vi "thermal_optical_capture_9.vi"() -> ()   [LabVIEW 2025]
panel:
  out "Times between Frames":u32
  in  "STOP ACQUISITION":bool
  out "File Name Out":string
  in  "File Path":string="C:\\Digambar\\Metal_thin_wall\\Optical_images\\Optical_images"
  out "Optical Preview":T1(plugin-control)
  in  "Focus":dbl(slide) scale=0.0..100.0
  out "Thermal Frame Out":string
  in  "Thermal Output Folder":path
  in  "thermal capture interval (s)":dbl
  in  "Flag Button":bool
  in  "Stop & Save":bool
  in  "Record":bool
  # "(1) Run VI"
  # "(2) After thermal camera calibration message (in terminal), press START"
  # "(3) Stop & Save"
  # "THERMAL CONTROLS"
  # "(Enter \"28\")"
  # "Thermal Record"
  # "OPTICAL CONTROLS"
  # "(must be an empty folder)"
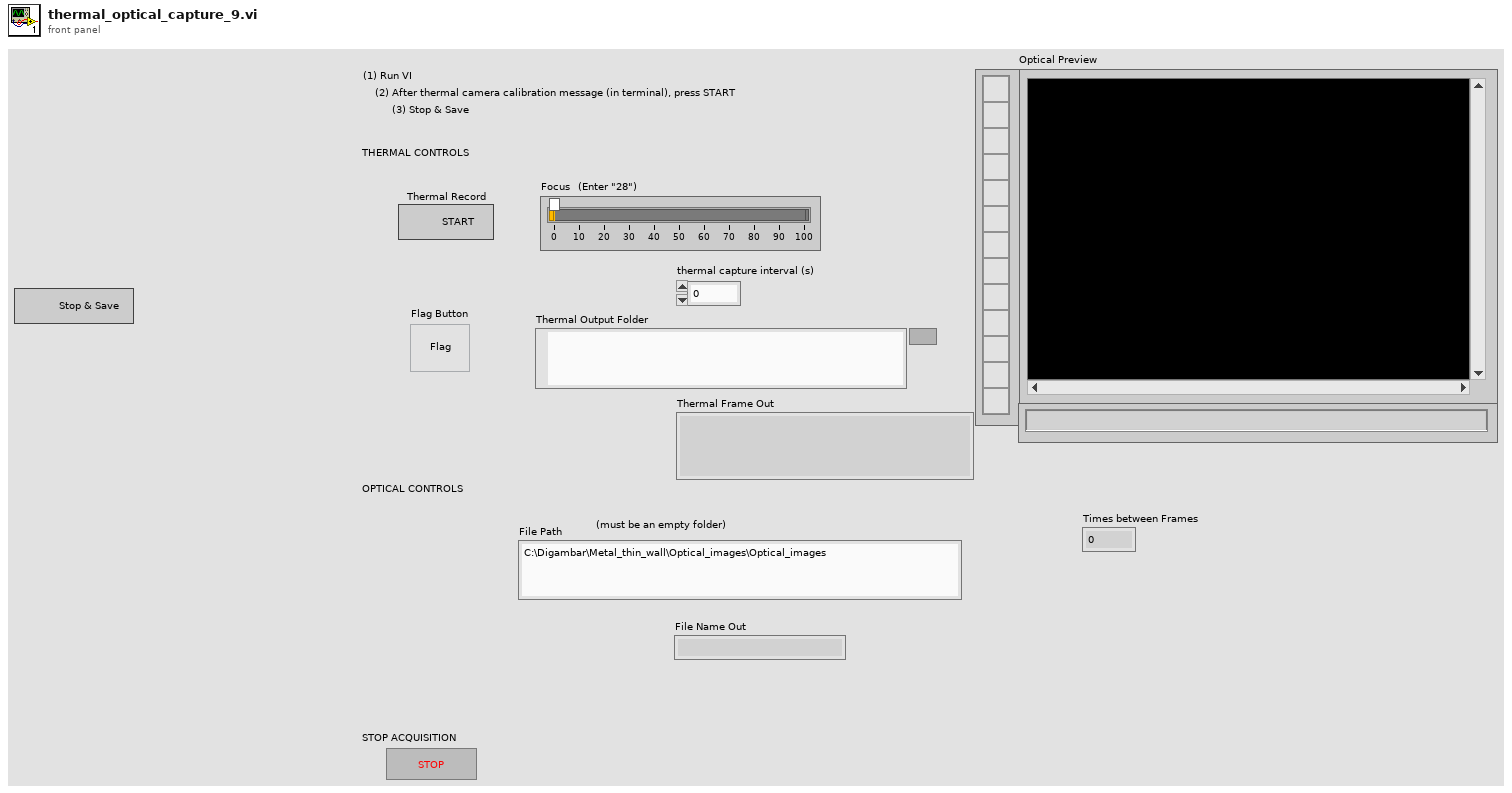
[diagram p1: front panel]
types:
  T1 = typedef "IMAQ Image.ctl" = refnum<image>
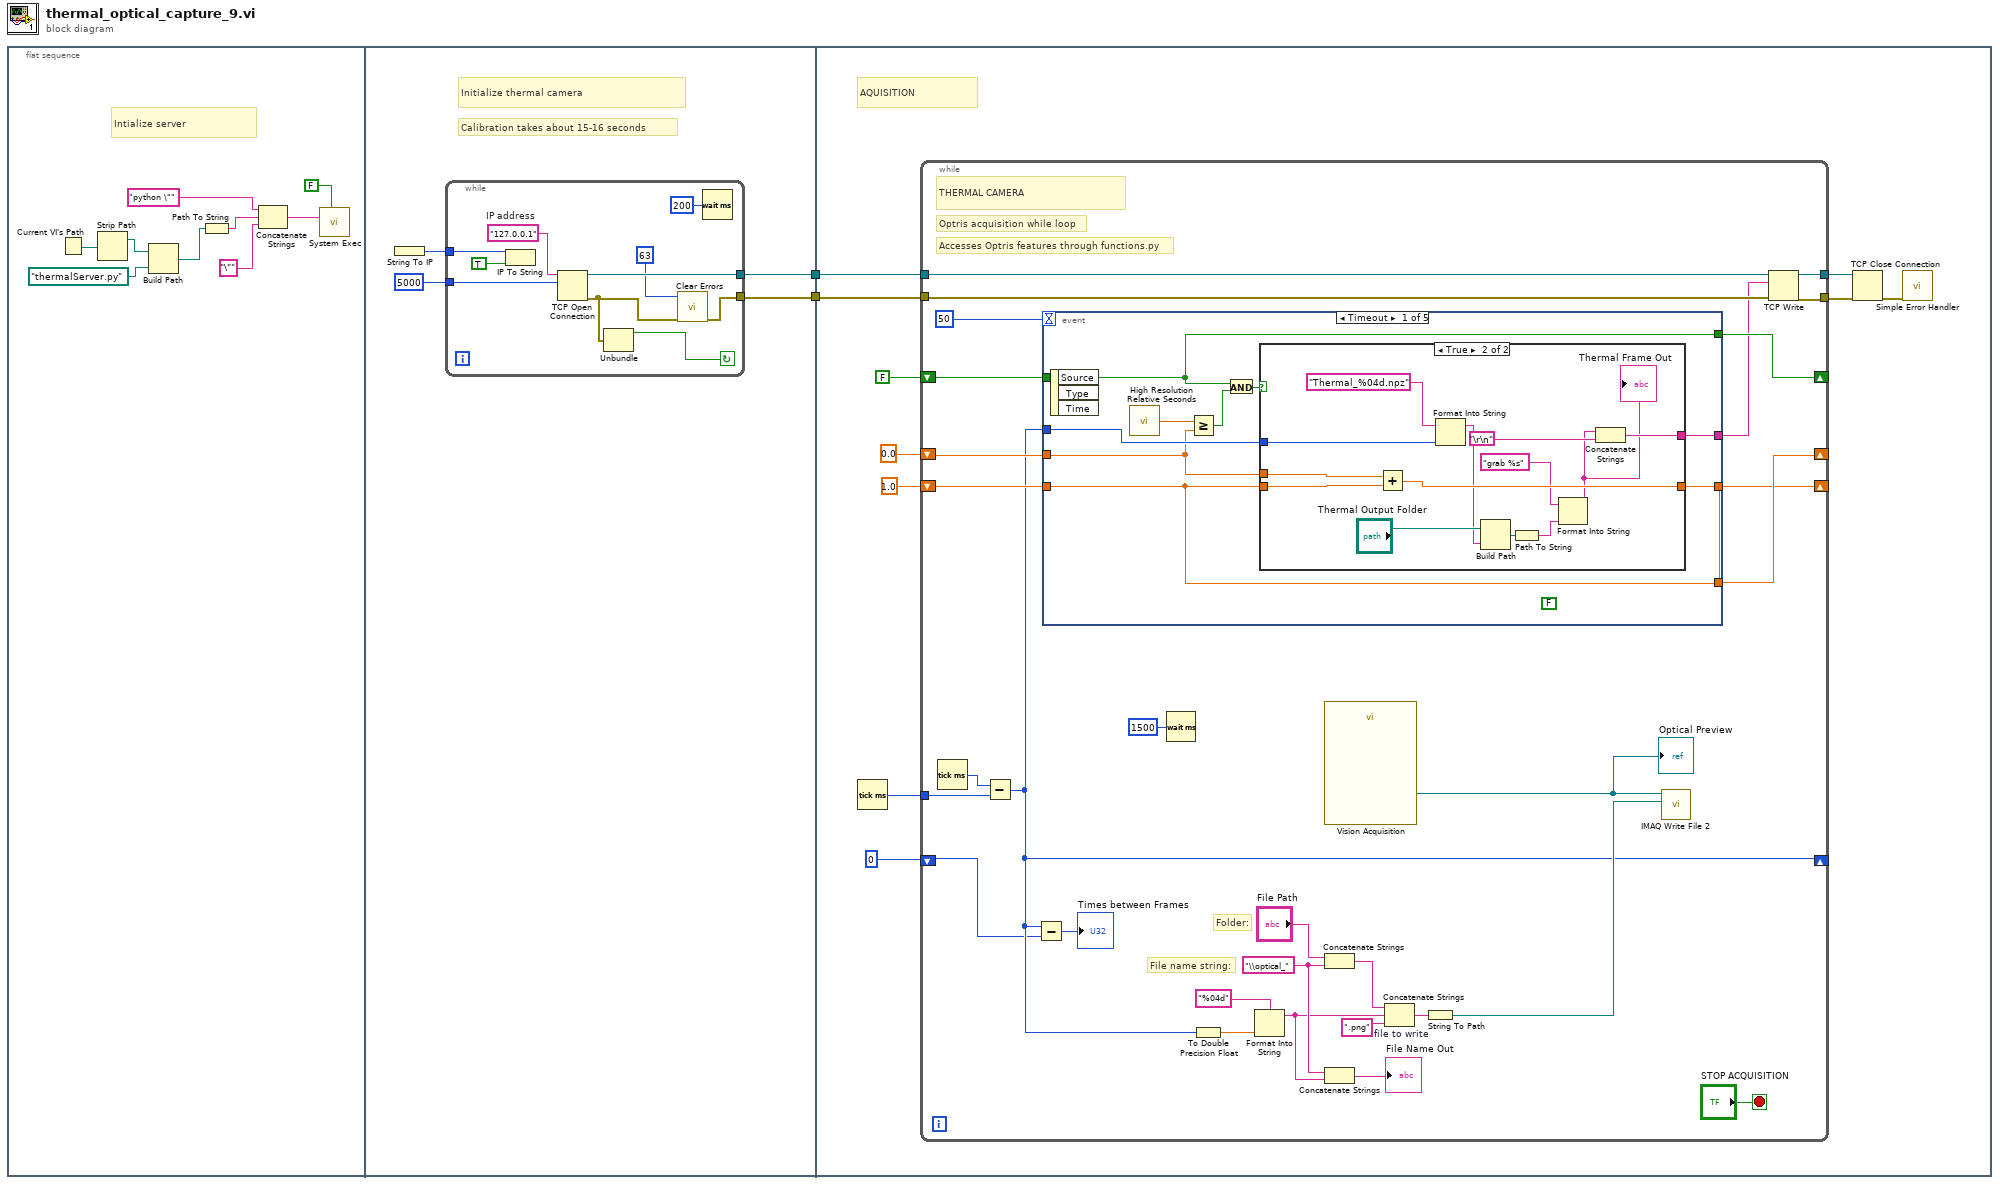
[diagram p0: block diagram]
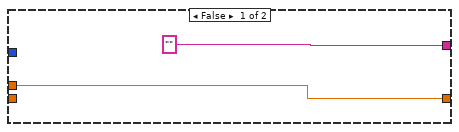
[diagram p2: hidden frame]
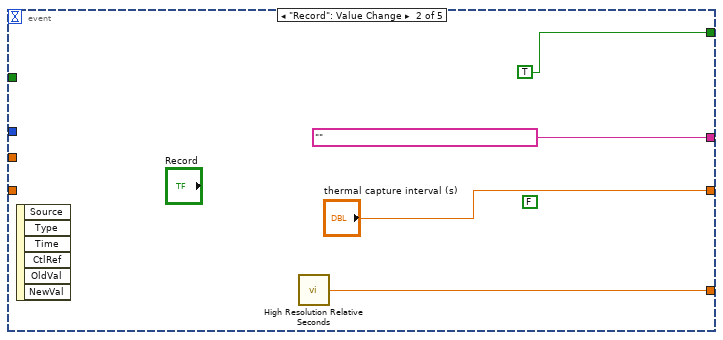
[diagram p3: hidden frame]
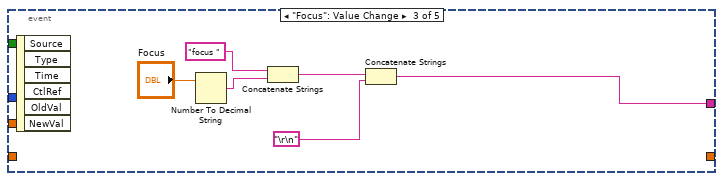
[diagram p4: hidden frame]
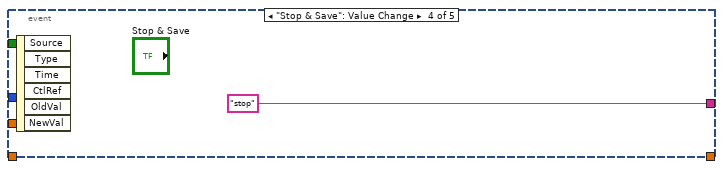
[diagram p5: hidden frame]
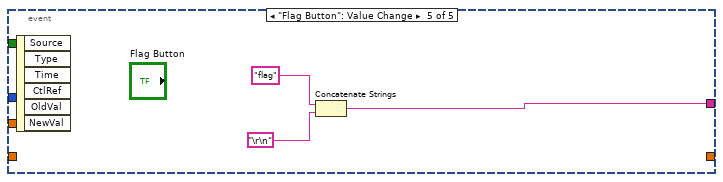
[diagram p6: hidden frame]
diagram:
  n1 = flat-sequence {
    tunnel: [w13] -> w2
    tunnel: [w12] -> w1
    tunnel: w1 -> [w32]
    tunnel: w2 -> [w31]
    frame #0 {
      # "Intialize server"
      n2 = Current VI's Path() -> (path=w6:path)
      n3 = Strip Path(path=w6) -> (stripped path=w7:path)  [unwired: 1 out]
      n4 = Build Path(base path=w7, name or relative path=path "thermalServer.py") -> (appended path=w4:path)
      n5 = Path To String(path=w4) -> (string=w10:string)
      n6 = Concatenate Strings("python \"" ("string"), w10, "\"" ("string")) -> (w9:string)
      n7 = call <vilib>:"System Exec.vi"("wait until completion? (T)"=FALSE, "command line"=w9) -> ()  [unwired: 6 in, 4 out]
    }
    frame #1 {
      # "Initialize thermal camera"
      # "Calibration takes about 15-16 seconds"
      n8 = String To IP() -> (0:w15:u32)  [unwired: 1 in]
      n9 = while {
        tunnel: [w20] -> w13
        tunnel: [w25] -> w12
        tunnel: w15 -> [w24]
        tunnel: u16 5000 ("remote port or service name") -> [w22]
        stop <- w17 continue-if-true
        w16 = "127.0.0.1"  # IP address
        n10 = IP To String(1:TRUE ("dot notation? (F)"), 2:w24) -> ()  [unwired: 1 out]
        n11 = TCP Open Connection(address=w16, remote port or service name=w22) -> (connection ID=w25:refnum<k5>, error out=w21:errorcluster)  [unwired: 3 in]
        n12 = Unbundle(w21) -> ("status"=w17:bool)  [unwired: 2 out]
        n13 = call <vilib>:"Clear Errors.vi"("error in (no error)"=w21, "specific error code to clear (0: all)"=63) -> ("error out"=w20:errorcluster)  [unwired: 4 in, 1 out]
        n14 = Wait (ms)(milliseconds to wait=u32 200) -> ()  [unwired: 1 out]
      }
    }
    frame #2 {
      # "AQUISITION"
      n15 = Tick Count (ms)() -> (millisecond timer value=w27:u32)
      n16 = while {
        tunnel: [w65] -> w33
        tunnel: [w64] -> w34
        tunnel: w32 -> [w63]
        tunnel: w31 -> [w62]
        shift-right: [w61] -> _
        shift-left: 0.0 -> [w57]
        shift-right: [w58] -> _
        shift-left: 1.0 -> [w55]
        shift-right: [w59] -> _
        shift-left: FALSE -> [w56]
        tunnel: w27 -> [w39]
        shift-right: [w38] -> _
        shift-left: u32 0 -> [w37]
        stop <- "STOP ACQUISITION" stop-if-true
        w48 = "\\optical_" ("string")
        # "Folder:"
        # "File name string:"
        # "THERMAL CAMERA"
        # "Optris acquisition while loop"
        # "Accesses Optris features through functions.py"
        n17 = Tick Count (ms)() -> (millisecond timer value=w40:u32)
        n18 = Subtract(x=w40, y=w39) -> (x-y=w38:u32)
        n19 = Subtract(x=w38, y=w37) -> (x-y=→"Times between Frames":u32)
        n20 = event shown="[0] Timeout" {
          selector: _ -> [_ _ _ _ _]
          dyn-events: _ -> [_ _ _ _ _]
          timeout: 50 -> [_ _ _ _ _]
          tunnel: [w70 "" w94 "stop" w103] -> w54
          tunnel: w38 -> [w71 _ _ _ _]
          tunnel: [w68 w93 _ _ _] -> w61
          tunnel: [w66 TRUE _ _ _] -> w59
          tunnel: [w67 "thermal capture interval (s)" _ _ _] -> w58
          tunnel: w57 -> [w69 _ _ _ _]
          tunnel: w56 -> [w66 _ _ _ _]
          tunnel: w55 -> [w67 _ _ _ _]
          event Timeout {
            (unwired) FALSE
            n21 = event-data() -> ()  [unwired: 1 in, 3 out]
            n22 = call <vilib>:"High Resolution Relative Seconds.vi"() -> ("relative seconds"=w74:dbl)
            n23 = Greater Or Equal?(x=w74, y=w69) -> (x >= y?=w73:bool)
            n24 = And(x=w66, y=w73) -> (x .and. y?=w72:bool)
            n25 = case shown="True" w72 {
              tunnel: w71 -> [_ w87]
              tunnel: ["" w88] -> w70
              tunnel: w69 -> [w75 w86]
              tunnel: w67 -> [_ w85]
              tunnel: [w75 w84] -> w68
              frame False {
              }
              frame True {
                n26 = Add(x=w86, y=w85) -> (x+y=w84:dbl)
                n27 = Format Into String(format string="Thermal_%04d.npz", w87) -> (resulting string=w79:string)  [unwired: 2 in, 1 out]
                n28 = Build Path(base path="Thermal Output Folder", name or relative path=w79) -> (appended path=w81:path)
                n29 = Path To String(path=w81) -> (string=w78:string)
                n30 = Format Into String(format string="grab %s", w78) -> (resulting string=w77:string)  [unwired: 2 in, 1 out]
                "Thermal Frame Out" <- w77
                n31 = Concatenate Strings(w77, "\r\n") -> (w88:string)
              }
            }
          }
          event "Record": Value Change {
            (unwired) FALSE
            n32 = event-data() -> ()  [unwired: 1 in, 6 out]
            n33 = call <vilib>:"High Resolution Relative Seconds.vi"() -> ("relative seconds"=w93:dbl)
          }
          event "Focus": Value Change {
            n34 = event-data() -> ()  [unwired: 1 in, 6 out]
            n35 = Number To Decimal String(number="Focus") -> (decimal integer string=w99:string)  [unwired: 1 in]
            n36 = Concatenate Strings("focus ", w99) -> (w96:string)
            n37 = Concatenate Strings(w96, "\r\n") -> (w94:string)
          }
          event "Stop & Save": Value Change {
            n38 = event-data() -> ()  [unwired: 1 in, 6 out]
          }
          event "Flag Button": Value Change {
            n39 = event-data() -> ()  [unwired: 1 in, 6 out]
            n40 = Concatenate Strings("flag", "\r\n") -> (w103:string)
          }
        }
        n41 = Wait (ms)(milliseconds to wait=u32 1500) -> ()  [unwired: 1 out]
        n42 = To Double Precision Float(number=w38) -> (double precision float=w46:dbl)
        n43 = Format Into String(format string="%04d" ("time format string (%c)"), w46) -> (resulting string=w44:string)  [unwired: 2 in, 1 out]
        n44 = call "Vision Acquisition"() -> ("Image Out"=w53:T1)  [unwired: 26 in, 1 out]
        "Optical Preview" <- w53
        n45 = Concatenate Strings("File Path", w48) -> (w49:string)
        n46 = Concatenate Strings(w48, w44) -> (→"File Name Out":string)
        n47 = Concatenate Strings "file to write"(w49, w44, ".png" ("string")) -> (w52:string)
        n48 = String To Path(string=w52) -> (path=w45:path)
        n49 = call-poly "IMAQ Write File 2"("File Path"=w45, "Image"=w53) -> ()  [unwired: 8 in, 2 out]
        n50 = TCP Write(connection ID=w63, data in=w54, error in (no error)=w62) -> (connection ID out=w64:refnum<k5>, error out=w65:errorcluster)  [unwired: 1 in, 1 out]
      }
      n51 = TCP Close Connection(connection ID=w34, error in (no error)=w33) -> (error out=w35:errorcluster)  [unwired: 1 in, 1 out]
      n52 = call <vilib>:"Simple Error Handler.vi"("error in (no error)"=w35) -> ()  [unwired: 4 in, 5 out]
    }
  }
